vi "Run All.vi"(8 "Error In":errorcluster) -> (0 "Error Out":errorcluster)   [LabVIEW 2017, in "Tests.lvlib" / "From Msgpack.lvlib"]
uses:
  From Msgpack.lvlib
  <vilib>/addons/_JKI Toolkits/Caraya/classes/Test/Test.lvclass
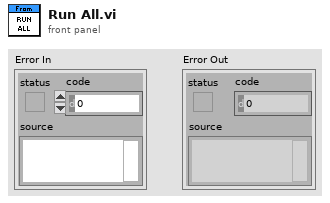
[diagram p1: front panel]
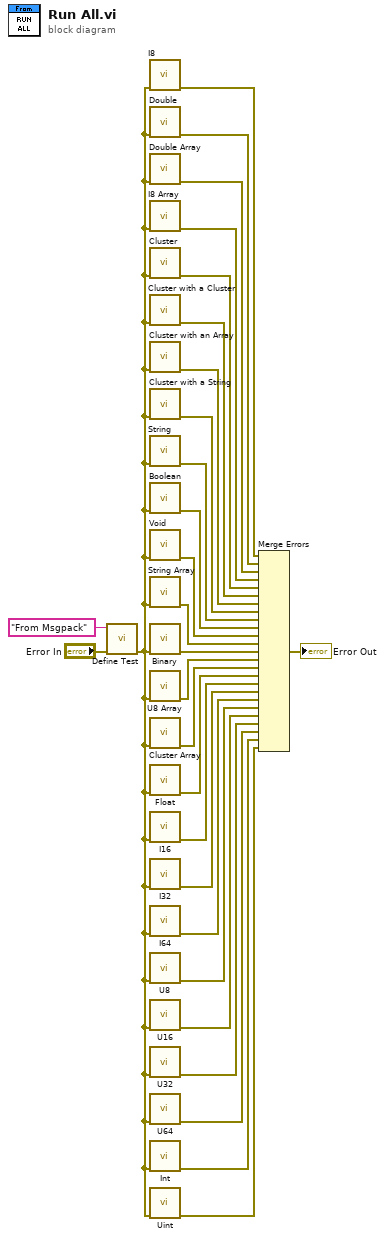
[diagram p0: block diagram]
diagram:
  n1 = call <vilib>:"Define Test.vi"("error in (no error)"="Error In", "Label (VI Title)"="From Msgpack") -> ("error out"=w2:errorcluster)  [unwired: 9 in]
  n2 = call "I8.vi"("Error In"=w2) -> ("Error Out"=w27:errorcluster)  [unwired: 10 in]
  n3 = call "Double.vi"("Error In"=w2) -> ("Error Out"=w25:errorcluster)  [unwired: 10 in]
  n4 = call "Double Array.vi"("Error In"=w2) -> ("Error Out"=w24:errorcluster)  [unwired: 10 in]
  n5 = call "I8 Array.vi"("Error In"=w2) -> ("Error Out"=w23:errorcluster)  [unwired: 10 in]
  n6 = call "Cluster.vi"("Error In"=w2) -> ("Error Out"=w22:errorcluster)  [unwired: 10 in]
  n7 = call "Cluster with a Cluster.vi"("Error In"=w2) -> ("Error Out"=w21:errorcluster)  [unwired: 10 in]
  n8 = call "Cluster with an Array.vi"("Error In"=w2) -> ("Error Out"=w20:errorcluster)  [unwired: 10 in]
  n9 = call "Cluster with a String.vi"("Error In"=w2) -> ("Error Out"=w19:errorcluster)  [unwired: 10 in]
  n10 = call "String.vi"("Error In"=w2) -> ("Error Out"=w18:errorcluster)  [unwired: 10 in]
  n11 = call "Boolean.vi"("Error In"=w2) -> ("Error Out"=w17:errorcluster)  [unwired: 10 in]
  n12 = call "Void.vi"("Error In"=w2) -> ("Error Out"=w16:errorcluster)  [unwired: 10 in]
  n13 = call "String Array.vi"("Error In"=w2) -> ("Error Out"=w15:errorcluster)  [unwired: 10 in]
  n14 = call "Binary.vi"("Error In"=w2) -> ("Error Out"=w14:errorcluster)  [unwired: 10 in]
  n15 = call "U8 Array.vi"("Error In"=w2) -> ("Error Out"=w13:errorcluster)  [unwired: 10 in]
  n16 = call "Cluster Array.vi"("Error In"=w2) -> ("Error Out"=w12:errorcluster)  [unwired: 10 in]
  n17 = call "Float.vi"("Error In"=w2) -> ("Error Out"=w11:errorcluster)  [unwired: 10 in]
  n18 = call "I16.vi"("Error In"=w2) -> ("Error Out"=w10:errorcluster)  [unwired: 10 in]
  n19 = call "I32.vi"("Error In"=w2) -> ("Error Out"=w9:errorcluster)  [unwired: 10 in]
  n20 = call "I64.vi"("Error In"=w2) -> ("Error Out"=w8:errorcluster)  [unwired: 10 in]
  n21 = call "U8.vi"("Error In"=w2) -> ("Error Out"=w7:errorcluster)  [unwired: 10 in]
  n22 = call "U16.vi"("Error In"=w2) -> ("Error Out"=w6:errorcluster)  [unwired: 10 in]
  n23 = call "U32.vi"("Error In"=w2) -> ("Error Out"=w5:errorcluster)  [unwired: 10 in]
  n24 = call "U64.vi"("Error In"=w2) -> ("Error Out"=w4:errorcluster)  [unwired: 10 in]
  n25 = call "Int.vi"("Error In"=w2) -> ("Error Out"=w3:errorcluster)  [unwired: 10 in]
  n26 = call "Uint.vi"("Error In"=w2) -> ("Error Out"=w1:errorcluster)  [unwired: 10 in]
  n27 = Merge Errors(w27, w25, w24, w23, w22, w21, w20, w19, w18, w17, w16, w15, w14, w13, w12, w11, w10, w9, w8, w7, w6, w5, w4, w3, w1) -> (→"Error Out":errorcluster)
